vi "SafetyStatus.vi"(0 "Universal Robot.lvclass in":refnum<class "Universal Robot.lvclass">, 5 "error in (no error)":errorcluster) -> (11 "safetyStatus out":T1, 14 "Universal Robot.lvclass out":refnum<class "Universal Robot.lvclass">, 19 "error out":errorcluster)   [LabVIEW 2019, in "Universal Robot.lvclass"]
uses:
  Universal Robot.lvclass
  SafetyStatus.ctl
  Universal Robot.lvclass/Universal Robot.ctl
  Client Interfaces/Dashboard Server/Dashboard Server.lvclass
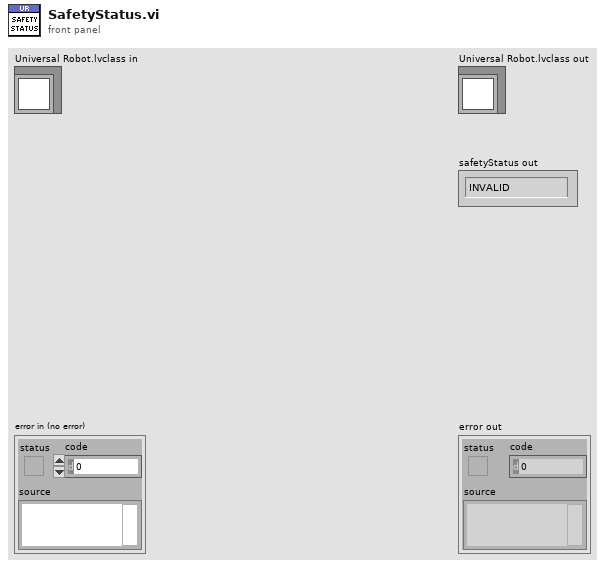
[diagram p1: front panel]
types:
  T1 = typedef "Universal Robot.lvclass/SafetyStatus.ctl" = enum16{"INVALID", "NORMAL", "REDUCED", "PROTECTIVE_STOP", "RECOVERY", "SAFEGUARD_STOP", "SYSTEM_EMERGENCY_STOP", "ROBOT_EMERGENCY_STOP", "VIOLATION", "FAULT", "AUTOMATIC_MODE_SAFEGAURD_STOP", "SYSTEM_THREE_POSITION_ENABLING_STOP"}
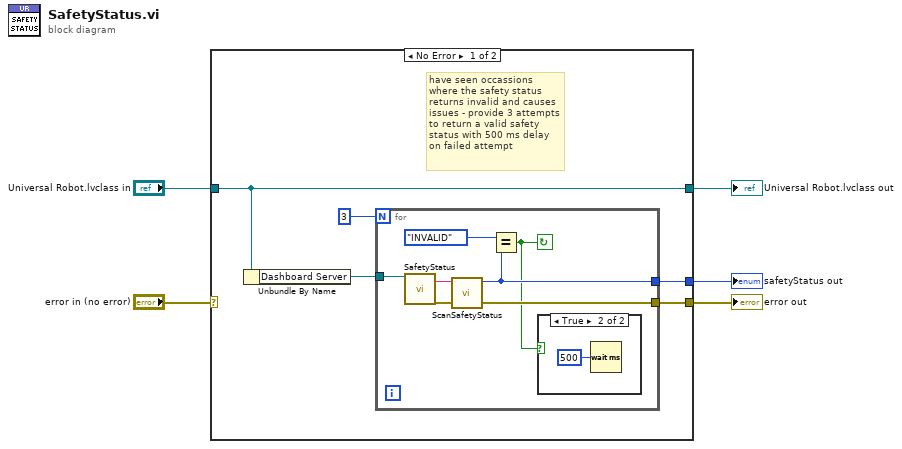
[diagram p0: block diagram]
diagram:
  n1 = case shown="No Error" "error in (no error)" {
    selector: "error in (no error)" -> [_ w19]
    tunnel: [w9 w19] -> w4
    tunnel: "Universal Robot.lvclass in" -> [w10 w18]
    tunnel: [w10 w18] -> w2
    tunnel: [w7 _] -> w1
    frame No Error {
      # "have seen occassions where the safety status returns invalid and causes issues - provide 3 attempts to return a valid safety status with 500 ms delay on failed attempt"
      n2 = Unbundle By Name(w10) -> ("Dashboard Server"=w8:refnum<class "Dashboard Server.lvclass">)
      n3 = for {
        N: 3 -> [_]
        tunnel: [w16] -> w9
        tunnel: w8 -> [w14]
        tunnel: [w13] -> w7
        stop <- w11 continue-if-true
        n4 = call-dynamic "SafetyStatus.vi"("DashboardServer in"=w14) -> ("safetyStatus"=w15:string, "error out"=w16:errorcluster)  [unwired: 16 in, 1 out]
        n5 = call "ScanSafetyStatus.vi"("safetyStatus in"=w15) -> ("safetyStatus out"=w13:T1)  [unwired: 10 in]
        n6 = Equal?(x=SafetyStatus."INVALID", y=w13) -> (x = y?=w11:bool)
        n7 = case shown="True" w11 {
          frame False {
          }
          frame True {
            n8 = Wait (ms)(milliseconds to wait=u32 500) -> ()  [unwired: 1 out]
          }
        }
      }
    }
    frame Error {
    }
  }
  "error out" <- w4
  "Universal Robot.lvclass out" <- w2
  "safetyStatus out" <- w1
